vi "REV Status.vi"() -> ()   [LabVIEW 2026]
uses:
  <vilib>/REVLibDriver/REVLibDriver.lvlib
  <vilib>/MRC/MrcLib.lvlib
  <vilib>/REV Custom Controls/Spark Output Control Type.ctl
  <vilib>/REVLibDriver/subvi/RevLibError.ctl
  <vilib>/REV Custom Controls/c_Spark_PeriodicStatus0.ctl
  <vilib>/REV Custom Controls/c_Spark_PeriodicStatus1.ctl
  <vilib>/REV Custom Controls/c_Spark_PeriodicStatus2.ctl
  <vilib>/REV Custom Controls/c_Spark_PeriodicStatus3.ctl
  <vilib>/REV Custom Controls/c_Spark_PeriodicStatus4.ctl
  <vilib>/REV Custom Controls/c_Spark_PeriodicStatus5.ctl
  <vilib>/REV Custom Controls/c_Spark_PeriodicStatus6.ctl
  <vilib>/REV Custom Controls/c_Spark_PeriodicStatus7.ctl
  <vilib>/REV Custom Controls/c_Spark_PeriodicStatus8.ctl
  <vilib>/REV Custom Controls/c_Spark_PeriodicStatus9.ctl
panel:
  out "s9":T1
  out "s8":T2
  out "s7":T3
  out "s6":T4
  out "function return 10":T5
  out "function return 9":T5
  out "function return 8":T5
  out "function return 6":T5
  out "s5":T6
  out "s4":T7
  out "s3":T8
  out "s2":T9
  out "s1":T10
  out "function return 7":T5
  out "s0":T11
  out "function return 5":T5
  out "function return 4":T5
  out "function return 3":T5
  out "function return 2":T5
  out "function return":T5
  in  "Setpoint":dbl(slide) scale=-1.0..1.0
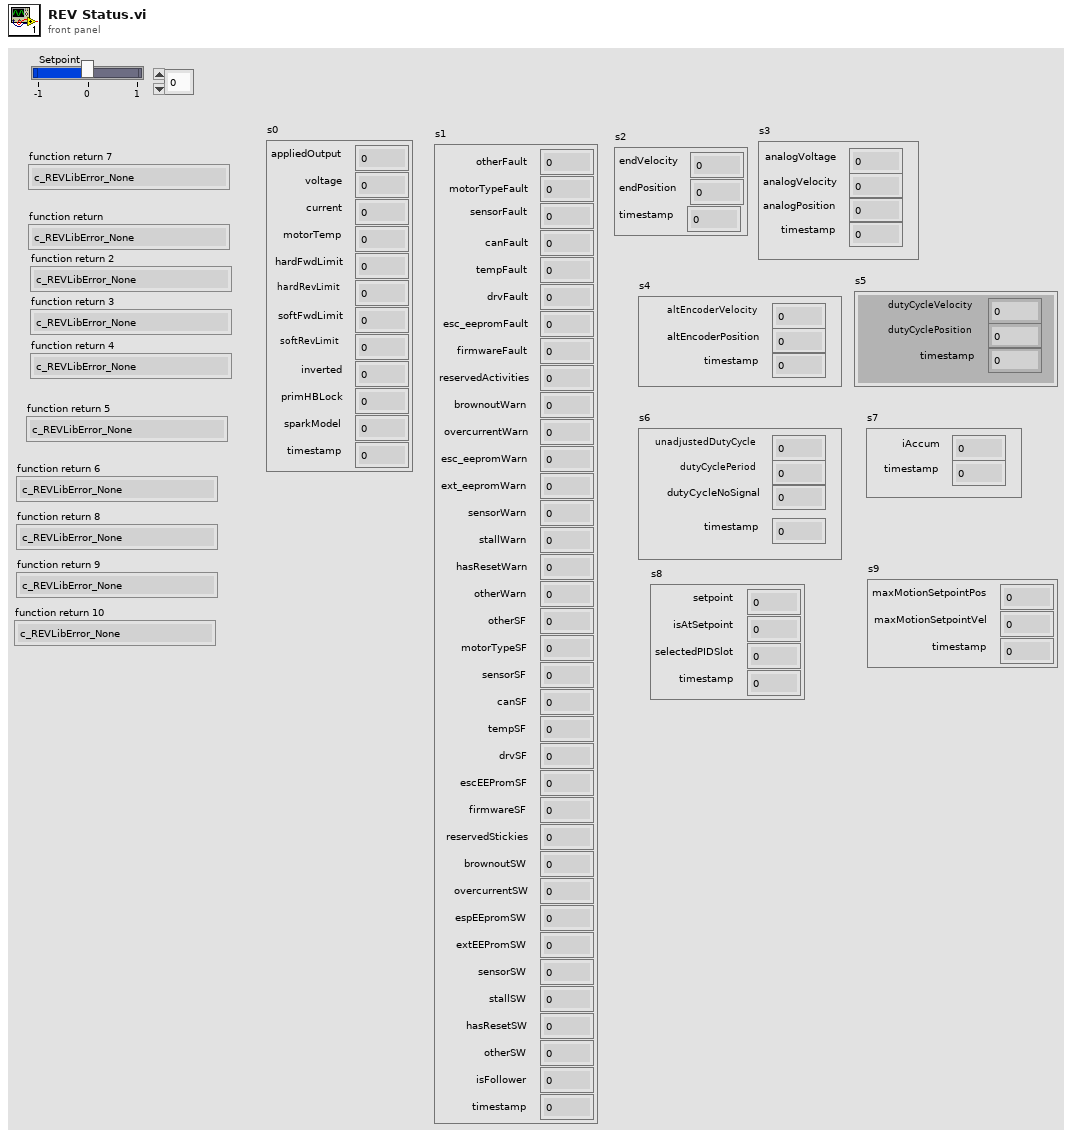
[diagram p1: front panel]
types:
  T1 = typedef "REVLibDriver.lvlib/c_Spark_PeriodicStatus9.ctl" = cluster{"maxMotionSetpointPos":sgl, "maxMotionSetpointVel":sgl, "timestamp":u64}
  T2 = typedef "REVLibDriver.lvlib/c_Spark_PeriodicStatus8.ctl" = cluster{"setpoint":sgl, "isAtSetpoint":u8, "selectedPIDSlot":u8, "timestamp":u64}
  T3 = typedef "REVLibDriver.lvlib/c_Spark_PeriodicStatus7.ctl" = cluster{"iAccum":sgl, "timestamp":u64}
  T4 = typedef "REVLibDriver.lvlib/c_Spark_PeriodicStatus6.ctl" = cluster{"unadjustedDutyCycle":sgl, "dutyCyclePeriod":sgl, "dutyCycleNoSignal":u8, "timestamp":u64}
  T5 = typedef "REVLibDriver.lvlib/RevLibError.ctl" = enum16{"c_REVLibError_None", "c_REVLibError_General", "c_REVLibError_CANTimeout", "c_REVLibError_NotImplemented", "c_REVLibError_HAL", "c_REVLibError_CantFindFirmware", "c_REVLibError_FirmwareTooOld", "c_REVLibError_FirmwareTooNew", "c_REVLibError_ParamInvalidID", "c_REVLibError_ParamMismatchType", "c_REVLibError_ParamAccessMode", "c_REVLibError_ParamInvalid", "c_REVLibError_ParamNotImplementedDeprecated", "c_REVLibError_FollowConfigMismatch", "c_REVLibError_Invalid", "c_REVLibError_SetpointOutOfRange", "c_REVLibError_Unknown", "c_REVLibError_CANDisconnected", "c_REVLibError_DuplicateCANId", "c_REVLibError_InvalidCANId", "c_REVLibError_SparkMaxDataPortAlreadyConfiguredDifferently", "c_REVLibError_SparkFlexBrushedWithoutDock", "c_REVLibError_InvalidBrushlessEncoderConfiguration", "c_REVLibError_FeedbackSensorIncompatibleWithDataPortConfig", "c_REVLibError_ParamInvalidChannel", "c_REVLibError_ParamInvalidValue", "c_REVLibError_CannotPersistParametersWhileEnabled", "c_REVLibError_NotReadyToReceiveCommand", "c_REVLibError_NumCodes"}
  T6 = typedef "REVLibDriver.lvlib/c_Spark_PeriodicStatus5.ctl" = cluster{"dutyCycleVelocity":sgl, "dutyCyclePosition":sgl, "timestamp":u64}
  T7 = typedef "REVLibDriver.lvlib/c_Spark_PeriodicStatus4.ctl" = cluster{"altEncoderVelocity":sgl, "altEncoderPosition":sgl, "timestamp":u64}
  T8 = typedef "REVLibDriver.lvlib/c_Spark_PeriodicStatus3.ctl" = cluster{"analogVoltage":sgl, "analogVelocity":sgl, "analogPosition":sgl, "timestamp":u64}
  T9 = typedef "REVLibDriver.lvlib/c_Spark_PeriodicStatus2.ctl" = cluster{"endVelocity":sgl, "endPosition":sgl, "timestamp":u64}
  T10 = typedef "REVLibDriver.lvlib/c_Spark_PeriodicStatus1.ctl" = cluster{"otherFault":u8, "motorTypeFault":u8, "sensorFault":u8, "canFault":u8, "tempFault":u8, "drvFault":u8, "esc_eepromFault":u8, "firmwareFault":u8, "reservedActivities":u8, "brownoutWarn":u8, "overcurrentWarn":u8, "esc_eepromWarn":u8, "ext_eepromWarn":u8, "sensorWarn":u8, "stallWarn":u8, "hasResetWarn":u8, "otherWarn":u8, "otherSF":u8, "motorTypeSF":u8, "sensorSF":u8, "canSF":u8, "tempSF":u8, "drvSF":u8, "escEEPromSF":u8, "firmwareSF":u8, "reservedStickies":u8, "brownoutSW":u8, "overcurrentSW":u8, "espEEpromSW":u8, "extEEPromSW":u8, "sensorSW":u8, "stallSW":u8, "hasResetSW":u8, "otherSW":u8, "isFollower":u8, "timestamp":u64}
  T11 = typedef "REVLibDriver.lvlib/c_Spark_PeriodicStatus0.ctl" = cluster{"appliedOutput":sgl, "voltage":sgl, "current":sgl, "motorTemp":u8, "hardFwdLimit":u8, "hardRevLimit":u8, "softFwdLimit":u8, "softRevLimit":u8, "inverted":u8, "primHBLock":u8, "sparkModel":u8, "timestamp":u64}
  T12 = typedef "REVLibDriver.lvlib/REVSparkRefnum.ctl" = refnum<k20>
  T13 = typedef "REVLibDriver.lvlib/Spark Output Control Type.ctl" = enum16{"Percent VBus", "Velocity", "Voltage", "Position", "Current", "MAXMotion Position", "MAXMotion Velocity"}
  T14 = typedef "REVLibDriver.lvlib/c_Spark_handle.ctl" = cluster{"Pointer":u64}
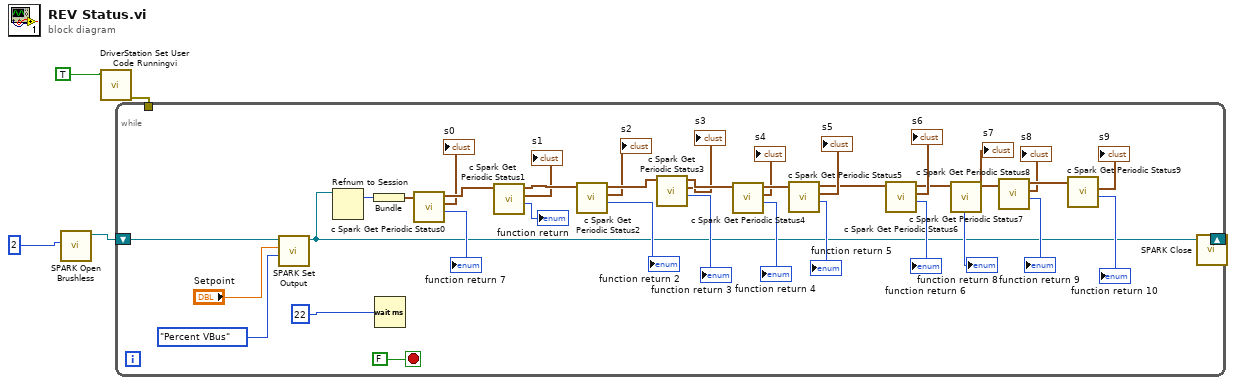
[diagram p0: block diagram]
diagram:
  n1 = call <vilib>:"SPARK Open Brushless.vi"("deviceId"=2) -> ("Spark refnum"=w4:T12)  [unwired: 9 in, 1 out]
  n2 = call <vilib>:"DriverStation Set User Code Runningvi.vi"("code ready for enable"=TRUE) -> ("error out"=w2:errorcluster)  [unwired: 10 in]
  n3 = while {
    shift-right: [w8] -> w1
    shift-left: w4 -> [w42]
    tunnel: w2 -> [_]
    stop <- FALSE stop-if-true
    n4 = call <vilib>:"SPARK Set Output.vi"("Control Mode"=Spark_Output_Control_Type."Percent VBus", "Setpoint"="Setpoint", "Spark refnum"=w42) -> ("Spark refnum"=w8:T12)  [unwired: 7 in, 1 out]
    n5 = Refnum to Session(7:w8) -> (3:w7:u64)  [unwired: 1 in, 1 out]
    n6 = Bundle("Session"=w7) -> (w6:cluster{"Session":u64})  [unwired: 1 in]
    n7 = Wait (ms)(milliseconds to wait=u32 22) -> ()  [unwired: 1 out]
    n8 = call <vilib>:"c Spark Get Periodic Status0.vi"("handle"=w6) -> ("function return"=→"function return 7":T5, "c_Spark_PeriodicStatus0"=→"s0":T11, "handle out"=w29:T14)  [unwired: 7 in, 1 out]
    n9 = call <vilib>:"c Spark Get Periodic Status1.vi"("handle"=w29) -> ("function return"=→"function return":T5, "spart_status_1"=→"s1":T10, "handle out"=w37:T14)  [unwired: 7 in, 1 out]
    n10 = call <vilib>:"c Spark Get Periodic Status2.vi"("handle"=w37) -> ("function return"=→"function return 2":T5, "c_Spark_PeriodicStatus2"=→"s2":T9, "handle out"=w36:T14)  [unwired: 7 in, 1 out]
    n11 = call <vilib>:"c Spark Get Periodic Status3.vi"("handle"=w36) -> ("function return"=→"function return 3":T5, "c_Spark_PeriodicStatus3"=→"s3":T8, "handle out"=w35:T14)  [unwired: 7 in, 1 out]
    n12 = call <vilib>:"c Spark Get Periodic Status4.vi"("handle"=w35) -> ("function return"=→"function return 4":T5, "c_Spark_PeriodicStatus4"=→"s4":T7, "handle out"=w34:T14)  [unwired: 7 in, 1 out]
    n13 = call <vilib>:"c Spark Get Periodic Status5.vi"("handle"=w34) -> ("function return"=→"function return 5":T5, "c_Spark_PeriodicStatus5"=→"s5":T6, "handle out"=w21:T14)  [unwired: 7 in, 1 out]
    n14 = call <vilib>:"c Spark Get Periodic Status6.vi"("handle"=w21) -> ("function return"=→"function return 6":T5, "c_Spark_PeriodicStatus6"=→"s6":T4, "handle out"=w10:T14)  [unwired: 7 in, 1 out]
    n15 = call <vilib>:"c Spark Get Periodic Status7.vi"("handle"=w10) -> ("function return"=→"function return 8":T5, "c_Spark_PeriodicStatus7"=→"s7":T3, "handle out"=w20:T14)  [unwired: 7 in, 1 out]
    n16 = call <vilib>:"c Spark Get Periodic Status8.vi"("handle"=w20) -> ("function return"=→"function return 9":T5, "c_Spark_PeriodicStatus8"=→"s8":T2, "handle out"=w19:T14)  [unwired: 7 in, 1 out]
    n17 = call <vilib>:"c Spark Get Periodic Status9.vi"("handle"=w19) -> ("function return"=→"function return 10":T5, "c_Spark_PeriodicStatus9"=→"s9":T1)  [unwired: 7 in, 2 out]
  }
  n18 = call <vilib>:"SPARK Close.vi"("Spark refnum"=w1) -> ()  [unwired: 10 in, 1 out]
